vi "Test_MCP_Server.vi"(8 "error in (no error)":errorcluster) -> (0 "error out":errorcluster)   [LabVIEW 2020, in "MCP Server tests.lvlib"]
uses:
  MCP Server tests.lvlib
  fake tool add.vi
  fake_tool_say_hello.vi
  fake tool return error.vi
  fake tool broken vi.vi
  fake tool no inputs outputs.vi
  fake resource short string.vi
  fake resource long string.vi
  fake resource broken vi.vi
  fake prompt broken vi.vi
  fake prompt concatanate strings.vi
  fake tool no description.vi
  fake tool arrays.vi
  src/MCP Server/MCP Server.lvlib
  fake tool ignored.vi
  416cc145-bc65-4336-831b-dce381f7377e.vi
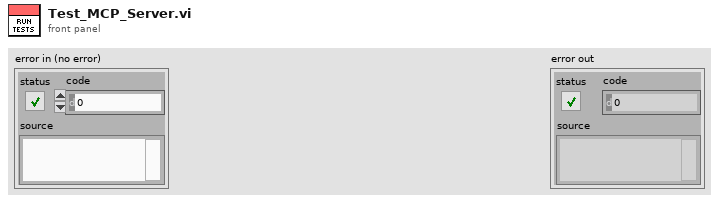
[diagram p1: front panel]
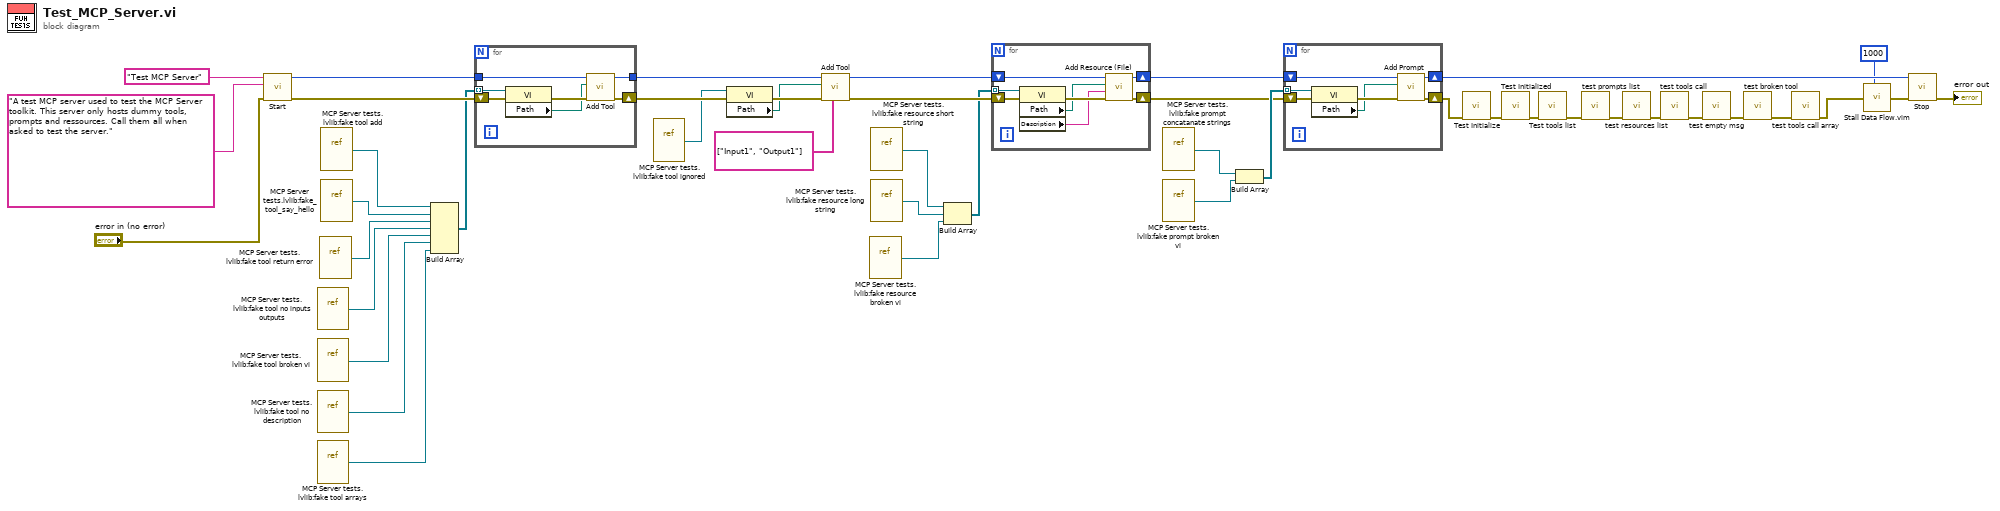
[diagram p0: block diagram]
diagram:
  n1 = call "Start.vi"("error in (no error)"="error in (no error)", "Description"="A test MCP server used to test the MCP Server toolkit. This server only hosts dummy tools, prompts and ressources. Call them all when asked to test the server.", "Name"="Test MCP Server") -> ("error out"=w44:errorcluster, "server id out"=w37:i32)  [unwired: 6 in, 1 out]
  n2 = vi-ref "MCP Server tests.lvlib:fake tool no inputs outputs.vi"() -> (w22:refnum<vi>)
  n3 = vi-ref "MCP Server tests.lvlib:fake tool broken vi.vi"() -> (w13:refnum<vi>)
  n4 = vi-ref "MCP Server tests.lvlib:fake tool no description.vi"() -> (w10:refnum<vi>)
  n5 = vi-ref "MCP Server tests.lvlib:fake tool arrays.vi"() -> (w5:refnum<vi>)
  n6 = vi-ref "MCP Server tests.lvlib:fake tool return error.vi"() -> (w39:refnum<vi>)
  n7 = vi-ref "MCP Server tests.lvlib:fake tool add.vi"() -> (w41:refnum<vi>)
  n8 = vi-ref "MCP Server tests.lvlib:fake_tool_say_hello.vi"() -> (w40:refnum<vi>)
  n9 = Build Array(w41, w40, w39, w22, w13, w10, w5) -> (w38:refnum<vi>[])
  n10 = for {
    shift-right: [w46] -> w36
    shift-left: w44 -> [w51]
    tunnel: w38 -> [w50] mode=indexing
    tunnel: w37 -> [w48]
    tunnel: [w47] -> w34
    n11 = property class="VI"(reference=w50, error in=w51) -> (error out=w49:errorcluster, "Path"=w45:path)  [unwired: 1 out]
    n12 = call "Add Tool.vi"("error in (no error)"=w49, "vi path"=w45, "server id"=w48) -> ("error out"=w46:errorcluster, "server id out"=w47:i32)  [unwired: 7 in]
  }
  n13 = vi-ref "MCP Server tests.lvlib:fake tool ignored.vi"() -> (w3:refnum<vi>)
  n14 = property class="VI"(reference=w3, error in=w36) -> (error out=w4:errorcluster, "Path"=w2:path)  [unwired: 1 out]
  n15 = call "Add Tool.vi"("Ignored"=string[] ["Input1", "Output1"], "error in (no error)"=w4, "vi path"=w2, "server id"=w34) -> ("error out"=w35:errorcluster, "server id out"=w33:i32)  [unwired: 6 in]
  n16 = vi-ref "MCP Server tests.lvlib:fake resource broken vi.vi"() -> (w9:refnum<vi>)
  n17 = vi-ref "MCP Server tests.lvlib:fake resource short string.vi"() -> (w31:refnum<vi>)
  n18 = vi-ref "MCP Server tests.lvlib:fake resource long string.vi"() -> (w32:refnum<vi>)
  n19 = Build Array(w31, w32, w9) -> (w30:refnum<vi>[])
  n20 = for {
    shift-right: [w58] -> w26
    shift-left: w35 -> [w57]
    shift-right: [w59] -> w27
    shift-left: w33 -> [w56]
    tunnel: w30 -> [w54] mode=indexing
    n21 = property class="VI"(reference=w54, error in=w57) -> (error out=w55:errorcluster, "Path"=w53:path, "Description"=w52:string)  [unwired: 1 out]
    n22 = call "Add Resource (File).vi"("error in (no error)"=w55, "description"=w52, "file path"=w53, "server id"=w56) -> ("error out"=w58:errorcluster, "server id out"=w59:i32)  [unwired: 6 in]
  }
  n23 = vi-ref "MCP Server tests.lvlib:fake prompt concatanate strings.vi"() -> (w28:refnum<vi>)
  n24 = vi-ref "MCP Server tests.lvlib:fake prompt broken vi.vi"() -> (w8:refnum<vi>)
  n25 = Build Array(w28, w8) -> (w29:refnum<vi>[])
  n26 = for {
    shift-right: [w65] -> w24
    shift-left: w26 -> [w64]
    shift-right: [w66] -> w25
    shift-left: w27 -> [w63]
    tunnel: w29 -> [w61] mode=indexing
    n27 = property class="VI"(reference=w61, error in=w64) -> (error out=w62:errorcluster, "Path"=w60:path)  [unwired: 1 out]
    n28 = call "Add Prompt.vi"("error in (no error)"=w62, "vi path"=w60, "server id"=w63) -> ("error out"=w65:errorcluster, "server id out"=w66:i32)  [unwired: 7 in]
  }
  n29 = call "Test Initialize.vi"("error in (no error)"=w24) -> ("error out"=w23:errorcluster)  [unwired: 9 in, 1 out]
  n30 = call "Test Initialized.vi"("error in (no error)"=w23) -> ("error out"=w21:errorcluster)  [unwired: 9 in, 1 out]
  n31 = call "Test tools list.vi"("error in (no error)"=w21) -> ("error out"=w20:errorcluster)  [unwired: 9 in, 1 out]
  n32 = call "test prompts list.vi"("error in (no error)"=w20) -> ("error out"=w19:errorcluster)  [unwired: 9 in, 1 out]
  n33 = call "test resources list.vi"("error in (no error)"=w19) -> ("error out"=w18:errorcluster)  [unwired: 9 in, 1 out]
  n34 = call "test tools call.vi"("error in (no error)"=w18) -> ("error out"=w17:errorcluster)  [unwired: 9 in, 1 out]
  n35 = call "test empty msg.vi"("error in (no error)"=w17) -> ("error out"=w14:errorcluster)  [unwired: 9 in, 1 out]
  n36 = call "test broken tool.vi"("error in (no error)"=w14) -> ("error out"=w7:errorcluster)  [unwired: 9 in, 1 out]
  n37 = call "test tools call array.vi"("error in (no error)"=w7) -> ("error out"=w6:errorcluster)  [unwired: 9 in, 1 out]
  n38 = call "Stall Data Flow.vim"("value in"=w6, "milliseconds to wait"=u32 1000) -> ("value out"=w12:errorcluster)  [unwired: 1 out]
  n39 = call "Stop.vi"("error in (no error)"=w12, "id"=w25) -> ("error out"=→"error out":errorcluster)  [unwired: 9 in]
